vi "RT_lab8.vi"() -> ()   [LabVIEW 2025]
uses:
  states.ctl
panel:
  out "Elements Remaining":u32
  out "Waveform Graph":i16[][](graph)
  out "error out":errorcluster
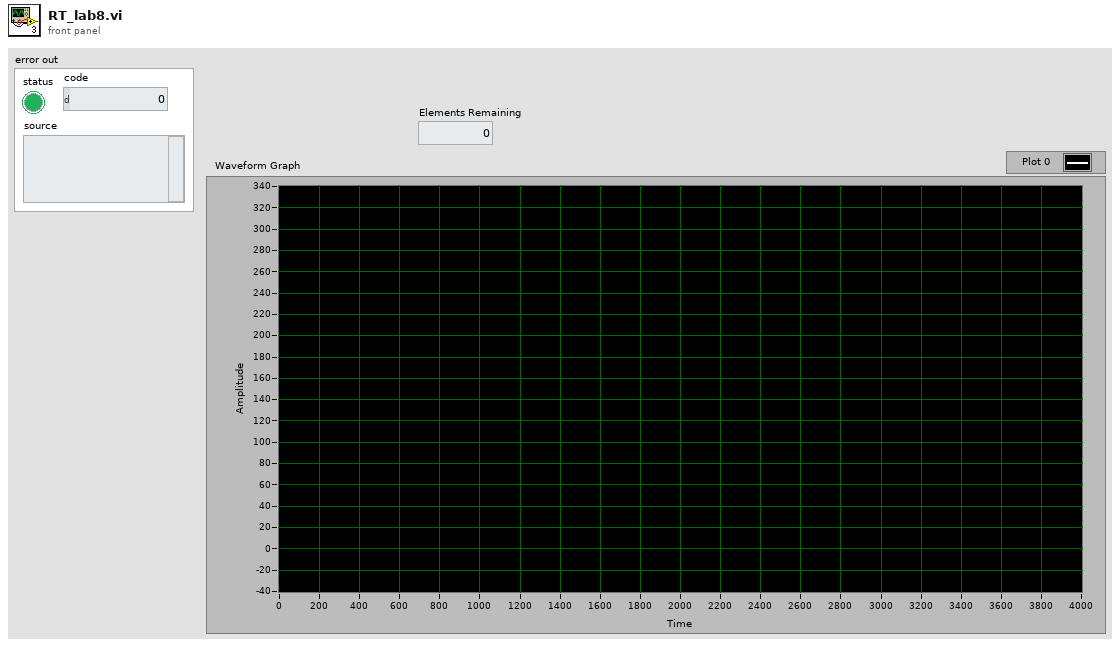
[diagram p1: front panel]
types:
  T1 = typedef "states.ctl" = enum16{"Run", "Connect"}
  T2 = typedef "RT_Cmd.ctl" = cluster{"command":T3, "parameters":T4}
  T3 = typedef "Command.ctl" = enum16{"threshold_config", "manual_trigger", "stop"}
  T4 = typedef "thresholds.ctl" = cluster{"Thr_X":i16, "Thr_Y":i16, "Thr_Z":i16}
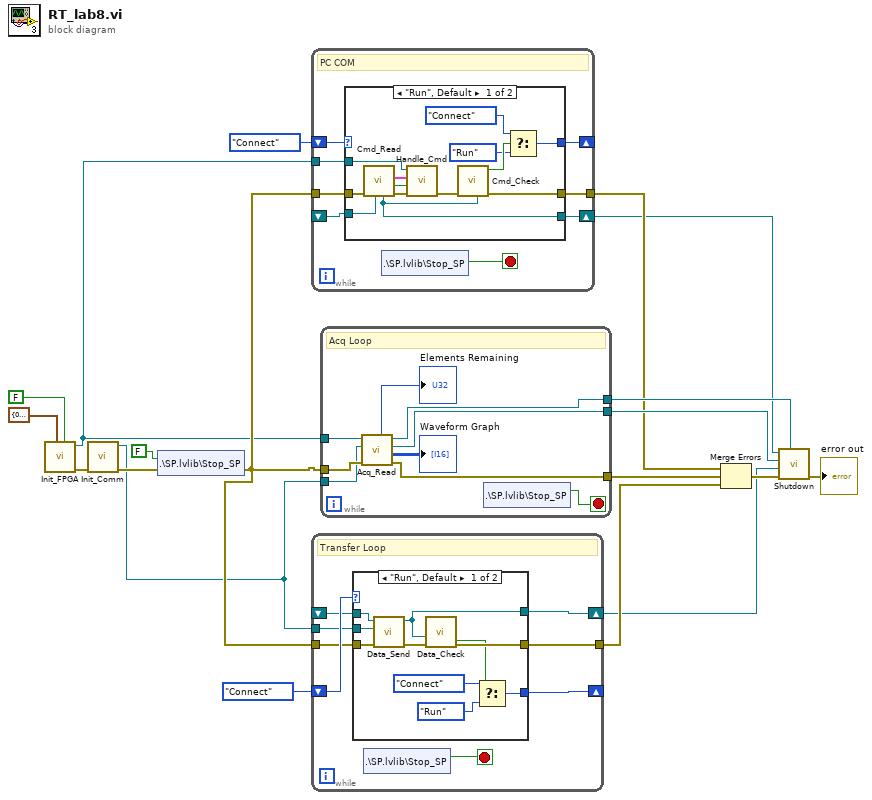
[diagram p0: block diagram]
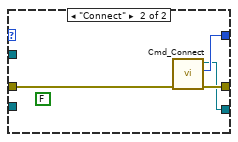
[diagram p2: hidden frame]
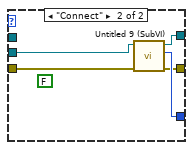
[diagram p3: hidden frame]
diagram:
  n1 = call "Init_FPGA.vi"("manual trigger"=FALSE, "Threshold"=cluster{"Thr_X":i16, "Thr_Y":i16, "Thr_Z":i16} {"Thr_X"=0, "Thr_Y"=0, "Thr_Z"=0}) -> ("error out"=w18:errorcluster, "FPGA VI Reference Out"=w8:refnum<k20>)  [unwired: 8 in]
  n2 = call "Init_Comm.vi"("error in"=w18) -> ("error out"=w14:errorcluster, "rt fifo ref out"=w11:refnum<k33>)  [unwired: 9 in]
  n3 = shared-variable ".\\SP.lvlib\\Stop_SP"(FALSE ("Stop_SP"), error in=w14) -> (error out=w12:errorcluster)
  n4 = while {
    tunnel: w12 -> [w26]
    tunnel: w8 -> [w25]
    shift-right: [w24] -> _
    shift-left: states."Connect" -> [w27]
    tunnel: [w23] -> w3
    shift-right: [w22] -> w1
    shift-left: _ -> [w21]
    stop <- w20 stop-if-true
    # "PC COM"
    n5 = case shown="\"Run\", Default" w27 {
      tunnel: w26 -> [w40 w44]
      tunnel: w25 -> [w38 _]
      tunnel: [w39 w43] -> w23
      tunnel: [w28 w42] -> w24
      tunnel: [w32 w41] -> w22
      tunnel: w21 -> [w33 _]
      frame "Run", Default {
        n6 = call "Cmd_Read.vi"("Refnum in"=w33, "error in (no error)"=w40) -> ("error out"=w35:errorcluster, "timed out?"=w36:bool, "data out"=w37:T2, "Refnum out"=w32:refnum<k21>)  [unwired: 6 in]
        n7 = call "Handle_Cmd.vi"("error in"=w35, "timed out?"=w36, "data IN"=w37, "FPGA VI Reference IN"=w38) -> ("error out"=w34:errorcluster)  [unwired: 6 in, 1 out]
        n8 = call "Cmd_Check.vi"("Refnum in"=w32, "error in (no error)"=w34) -> ("error out"=w39:errorcluster, "disconnected?"=w31:bool)  [unwired: 8 in]
        n9 = Select(t=states."Connect", s=w31, f=states."Run") -> (s? t:f=w28:T1)
      }
      frame "Connect" {
        (unwired) FALSE
        n10 = call "Cmd_Connect.vi"("error in (no error)"=w44) -> ("error out"=w43:errorcluster, "Enum"=w42:T1, "Refnum out"=w41:refnum<k21>)  [unwired: 8 in]
      }
    }
    n11 = shared-variable ".\\SP.lvlib\\Stop_SP"() -> (w20:bool)  [unwired: 1 in, 1 out]
  }
  n12 = while {
    tunnel: w11 -> [w49]
    tunnel: w12 -> [w48]
    shift-right: [w47] -> _
    shift-left: states."Connect" -> [w52]
    shift-right: [w51] -> w2
    shift-left: _ -> [w50]
    tunnel: [w46] -> w5
    stop <- w45 stop-if-true
    # "Transfer Loop"
    n13 = case shown="\"Run\", Default" w52 {
      tunnel: [w57 w67] -> w51
      tunnel: w50 -> [w60 _]
      tunnel: w49 -> [w62 w66]
      tunnel: w48 -> [w61 w65]
      tunnel: [w54 w64] -> w47
      tunnel: [w58 w63] -> w46
      frame "Run", Default {
        n14 = call "Data_Send.vi"("error in (no error)"=w61, "rt fifo ref in"=w62, "Refnum in"=w60) -> ("error out"=w59:errorcluster, "Refnum out"=w57:refnum<k21>)  [unwired: 7 in]
        n15 = call "Data_Check.vi"("error in (no error)"=w59, "Refnum in"=w57) -> ("error out"=w58:errorcluster, "disconnected?"=w56:bool)  [unwired: 8 in]
        n16 = Select(t=states."Connect", s=w56, f=states."Run") -> (s? t:f=w54:T1)
      }
      frame "Connect" {
        (unwired) FALSE ("Stop?")
        n17 = call "Untitled 9 (SubVI).vi"("error in (no error)"=w65, "Refnum in"=w66) -> ("error out"=w63:errorcluster, "Enum"=w64:T1, "Refnum out"=w67:refnum<k21>)  [unwired: 7 in]
      }
    }
    n18 = shared-variable ".\\SP.lvlib\\Stop_SP"() -> (w45:bool)  [unwired: 1 in, 1 out]
  }
  n19 = while {
    tunnel: w8 -> [w76]
    tunnel: w12 -> [w75]
    tunnel: [w74] -> w16
    tunnel: [w72] -> w4
    tunnel: w11 -> [w73]
    tunnel: [w71] -> w15
    stop <- w70 stop-if-true
    # "Acq Loop"
    n20 = call "Acq_Read.vi"("error in (no error)"=w75, "rt fifo ref in"=w73, "Refnum in"=w76) -> ("error out"=w72:errorcluster, "Array"=→"Waveform Graph":i16[][], "rt fifo ref out"=w71:refnum<k33>, "Refnum out"=w74:refnum<k20>, "Elements Remaining"=→"Elements Remaining":u32)  [unwired: 4 in]
    n21 = shared-variable ".\\SP.lvlib\\Stop_SP"() -> (w70:bool)  [unwired: 1 in, 1 out]
  }
  n22 = Merge Errors(w3, w4, w5) -> (w17:errorcluster)
  n23 = call "Shutdown.vi"("Refnum out 3"=w16, "error in (no error)"=w17, 9:"Refnum in"=w2, "rt fifo ref in"=w15, 11:"Refnum in"=w1) -> ("error out"=→"error out":errorcluster)  [unwired: 6 in]
